vi "Read Environment Variable.vi"(8 "error in":errorcluster, 11 "Variable":string) -> (0 "error out":errorcluster, 3 "Value":string)   [LabVIEW 2026]
doc: "Reads an environment variable value on Windows or Linux after validating the variable name. Returns an error for invalid names and otherwise uses a platform-specific shell command through System Exec.vi."
uses:
  <vilib>/regexp/Match Regular Expression.xnode
  <vilib>/Utility/error.llb/Trim Whitespace (string).vi
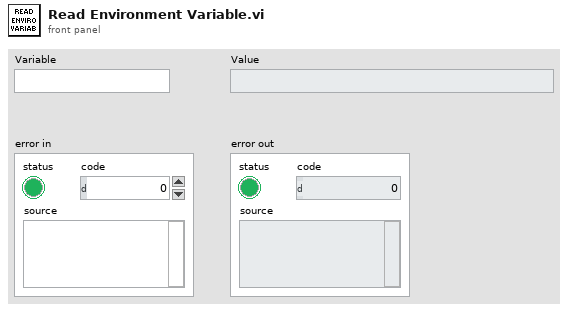
[diagram p1: front panel]
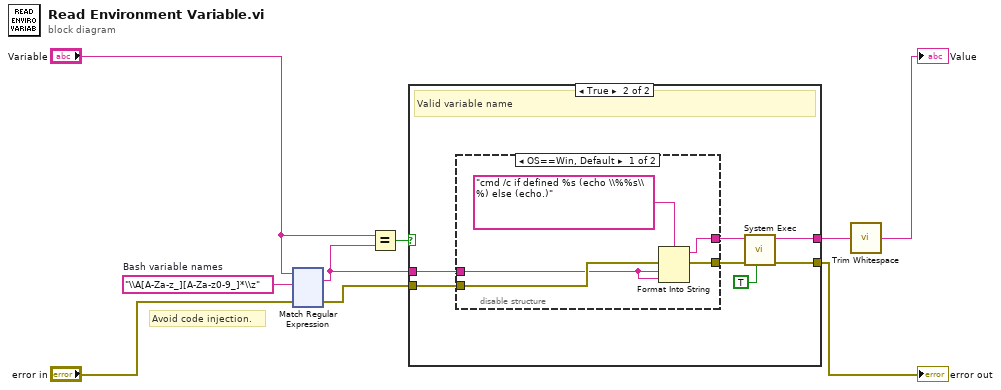
[diagram p0: block diagram]
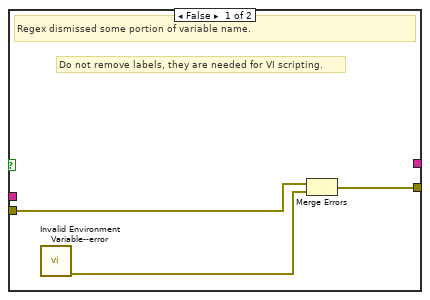
[diagram p2: hidden frame]
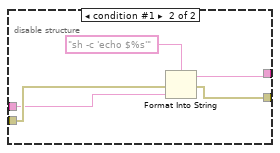
[diagram p3: hidden frame]
diagram:
  w6 = "\\A[A-Za-z_][A-Za-z0-9_]*\\z"  # Bash variable names
  # "Avoid code injection."
  n1 = xnode "Match Regular Expression"("input string"="Variable", "regular expression"=w6, "error in"="error in") -> ("whole match"=w4:string, "error out"=w7:errorcluster)  [unwired: 3 in, 3 out]
  n2 = Equal?(x="Variable", y=w4) -> (x = y?=w3:bool)
  n3 = case shown="True" w3 {
    tunnel: [w11 w18] -> w9
    tunnel: w7 -> [w10 w17]
    tunnel: [_ w14] -> w2
    tunnel: w4 -> [_ w13]
    frame False {
      # "Do not remove labels, they are needed for VI scripting."
      # "Regex dismissed some portion of variable name."
      n4 = call "Invalid Environment Variable--error.vi"() -> ("error out"=w12:errorcluster)  [unwired: 11 in]
      n5 = Merge Errors(w10, w12) -> (w11:errorcluster)
    }
    frame True {
      # "Valid variable name"
      n6 = disable-structure shown="OS==Win, Default" {
        disable-tunnel: w13 -> [w20 w26]
        disable-tunnel: w17 -> [w24 w28]
        disable-tunnel: [w23 w29] -> w19
        disable-tunnel: [w22 w25] -> w15
        frame condition #0 (active) {
          n7 = Format Into String(format string="cmd /c if defined %s (echo \\%%s\\%) else (echo.)", error in=w24, w20, w20) -> (resulting string=w22:string, error out=w23:errorcluster)  [unwired: 1 in]
        }
        frame condition #1 {
          n8 = Format Into String(format string="sh -c 'echo $%s'", error in=w28, w26) -> (resulting string=w25:string, error out=w29:errorcluster)  [unwired: 1 in]
        }
      }
      n9 = call <vilib>:"System Exec.vi"("run minimized? (F)"=TRUE, "error in (no error)"=w19, "command line"=w15) -> ("error out"=w18:errorcluster, "standard output"=w14:string)  [unwired: 5 in, 2 out]
    }
  }
  "error out" <- w9
  n10 = call-poly <vilib>:"Trim Whitespace.vi"("string"=w2) -> ("trimmed string"=→"Value":string)  [unwired: 1 in]
